vi "Msg Output Terminals.vi"(10 "Terminals (Msg Output)":T1) -> (1 "Terminals (Read Msg Output)":T1, 2 "Terminals (Init Msg Output)":T1)   [LabVIEW 2020, in "_Rescript.lvlib" / "Msg.lvlib" / "Msg.lvclass"]
uses:
  Msg.lvclass
  Terminals.ctl
  _Rescript.lvlib
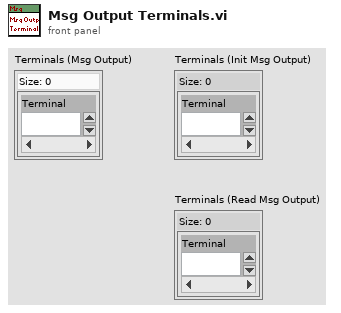
[diagram p1: front panel]
types:
  T1 = typedef "_Rescript.lvlib/Terminals.ctl" = set{i32}
  T2 = typedef "_Rescript.lvlib/Msg.lvlib/Msg.lvclass/Terminal Relation.ctl" = map{i32, i32}
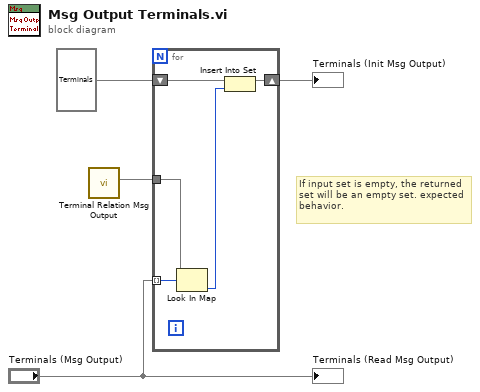
[diagram p0: block diagram]
diagram:
  # "If input set is empty, the returned set will be an empty set. expected behavior."
  n1 = call "Terminal Relation Msg Output.vi"() -> ("Terminal Relation (Msg Output)"=w1:T2)  [unwired: 11 in]
  n2 = for {
    tunnel: "Terminals (Msg Output)" -> [w8] mode=indexing
    tunnel: w1 -> [w9]
    shift-right: [w6] -> w3
    shift-left: T1 {} ("Terminals (Init Msg Output)") -> [w7]
    n3 = Look In Map(map=w9, key=w8) -> (value=w5:i32)  [unwired: 1 in, 1 out]
    n4 = Insert Into Set(10:w5, 11:w7) -> (3:w6:T1)  [unwired: 1 out]
  }
  "Terminals (Init Msg Output)" <- w3
  "Terminals (Read Msg Output)" <- "Terminals (Msg Output)"
